vi "Value Change.vi"(7 "objects":T1, 8 "error in":errorcluster, 11 "Multi Column Listbox in":refnum<class "Multi Column Listbox.lvclass">) -> (0 "error out":errorcluster, 2 "Update?":bool, 3 "Multi Column Listbox out":refnum<class "Multi Column Listbox.lvclass">)   [LabVIEW 2014, in "Table Manager.lvlib" / "Multi Column Listbox.lvclass"]
uses:
  Multi Column Listbox.lvclass
  Table Manager/object ref.ctl
  Configuration Editor/Classes/Engine Parent/Engine Parent Editor Node.lvclass
  Configuration Editor/Classes/Module editor node/module editor node.lvclass
  Table Manager/Table Manager.lvclass/Table Manager.ctl
  Multi Column Listbox.lvclass/Multi Column Listbox.ctl
  Line/Line.lvclass/Line.ctl
  Column/Column.lvclass/Column.ctl
  Table Manager/Read Line.vi
  Read Listbox.vi
  Table Manager/Read Index.vi
  Line/Read Columns.vi
  Line/Line.lvclass
  Column/Column.lvclass
  Table Manager/Table Manager.lvclass
  Table Manager.lvlib
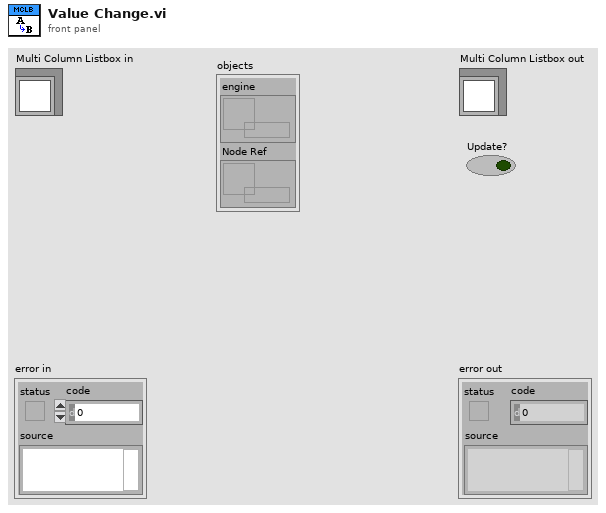
[diagram p1: front panel]
types:
  T1 = typedef "Table Manager.lvlib/Table Manager.lvclass/object ref.ctl" = cluster{"engine":refnum<data-value>, "Node Ref":refnum<data-value>}
  T2 = typedef "Table Manager.lvlib/Cell Change.ctl" = cluster{"row":i32, "col":i32, "old value":string, "new value":string}
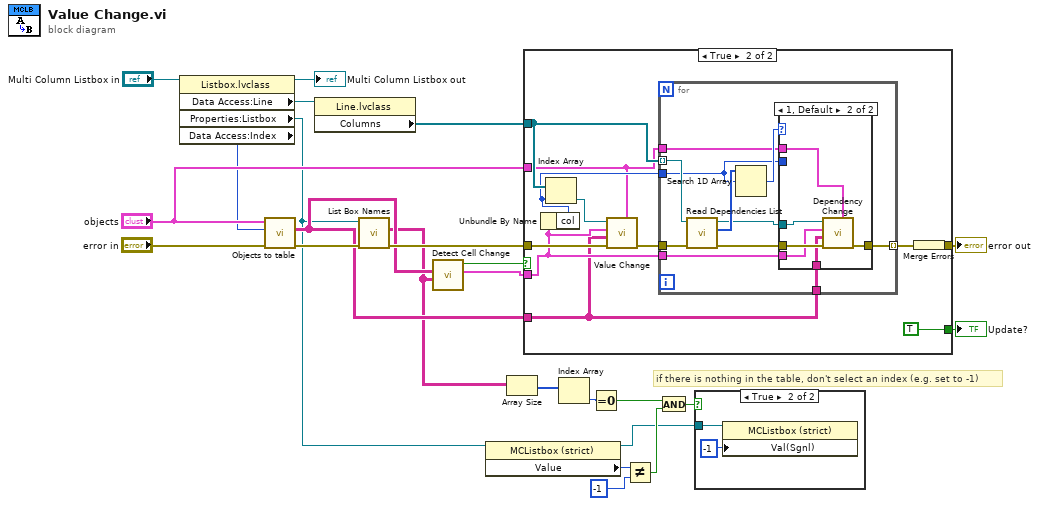
[diagram p0: block diagram]
diagram:
  # "if there is nothing in the table, don't select an index (e.g. set to -1)"
  n1 = property class="Listbox.lvclass"(reference="Multi Column Listbox in") -> (reference out=→"Multi Column Listbox out":refnum<class "Multi Column Listbox.lvclass">, "Data Access:Line"=w20:refnum<class "Line.lvclass">, "Properties:Listbox"=w1:refnum<vi>, "Data Access:Index"=w11:i32)  [unwired: 1 in, 1 out]
  n2 = call "Objects to table.vi"("error in (no error)"="error in", "Table Index"=w11, "object ref in"="objects") -> ("error out"=w24:errorcluster, "table"=w14:string[][])  [unwired: 6 in, 1 out]
  n3 = property class="Line.lvclass"(reference=w20) -> ("Columns"=w18:refnum<class "Column.lvclass">[])  [unwired: 1 in, 2 out]
  n4 = call "List Box Names.vi"("error in (no error)"=w24, "MulticolumnListbox in"=w1) -> ("error out"=w17:errorcluster, "ItemNames"=w2:string[][])  [unwired: 7 in, 1 out]
  n5 = call "Detect Cell Change.vi"("new values"=w2, "old values"=w14) -> ("Cluster"=w13:T2, "value change"=w15:bool)  [unwired: 6 in, 2 out]
  n6 = property class="MCListbox (strict)"(reference=w1) -> (reference out=w3:refnum<vi>, "Value"=w5:i32)  [unwired: 1 in, 1 out]
  n7 = Array Size(array=w2) -> (size(s)=w10:i32[])
  n8 = case shown="True" w15 {
    tunnel: [w25 w34] -> w19
    tunnel: w18 -> [_ w32]
    tunnel: w17 -> [w25 w31]
    tunnel: "objects" -> [_ w29]
    tunnel: w14 -> [_ w27]
    tunnel: w13 -> [_ w28]
    tunnel: [_ TRUE ("Update?")] -> w12
    frame False {
    }
    frame True {
      n9 = Unbundle By Name(w28) -> ("col"=w30:i32)
      n10 = Index Array(array=w32, index=w30) -> (element=w36:refnum<class "Column.lvclass">)
      n11 = call-dynamic "Value Change.vi"("object ref in"=w29, "error in (no error)"=w31, "old values"=w27, "Table Change"=w28, "Column in"=w36) -> ("error out"=w35:errorcluster)  [unwired: 5 in, 1 out]
      n12 = for {
        tunnel: w30 -> [w39]
        tunnel: w35 -> [w43]
        tunnel: [w47] -> w33 mode=indexing
        tunnel: w32 -> [w45] mode=indexing
        tunnel: w29 -> [w40]
        tunnel: w27 -> [w38]
        tunnel: w28 -> [w37]
        n13 = call "Read Dependencies List.vi"("error in (no error)"=w43, "Column in"=w45) -> ("error out"=w42:errorcluster, "Dependecies"=w46:i32[], "Column out"=w44:refnum<class "Column.lvclass">)  [unwired: 7 in]
        n14 = Search 1D Array(1D array=w46, element=w39) -> (index of element=w41:i32)  [unwired: 1 in]
        n15 = case shown="1, Default" w41 {
          tunnel: [w48 w54] -> w47
          tunnel: w42 -> [w48 w53]
          tunnel: w44 -> [_ w52]
          tunnel: w40 -> [_ w51]
          tunnel: w39 -> [_ _]
          tunnel: w38 -> [_ w50]
          tunnel: w37 -> [_ w49]
          frame -1 {
          }
          frame 1, Default {
            n16 = call-dynamic "Dependency Change.vi"("object ref in"=w51, "error in (no error)"=w53, "old values"=w50, "Table Change"=w49, "Column in"=w52) -> ("error out"=w54:errorcluster)  [unwired: 5 in, 1 out]
          }
        }
      }
      n17 = Merge Errors(w33) -> (w34:errorcluster)
    }
  }
  "error out" <- w19
  "Update?" <- w12
  n18 = Index Array(array=w10) -> (element=w9:i32)  [unwired: 1 in]
  n19 = Equal To 0?(x=w9) -> (x = 0?=w8:bool)
  n20 = Not Equal?(x=w5, y=-1) -> (x != y?=w6:bool)
  n21 = And(x=w8, y=w6) -> (x .and. y?=w7:bool)
  n22 = case shown="True" w7 {
    tunnel: w3 -> [_ w55]
    frame False {
    }
    frame True {
      n23 = property class="MCListbox (strict)"(reference=w55, "Val(Sgnl)"=-1) -> ()  [unwired: 1 in, 2 out]
    }
  }
